vi "Calculation.vi"(0 "Current(i)":dbl, 5 "Voltage(v)":dbl, 7 "Thickness Of Specimen(l)":dbl, 9 "Area of specimen(m2)":dbl, 11 "UPPER(Th-Tc)":dbl, 12 "error constant":errorcluster, 13 "LOWER(Th-Tc)":dbl) -> (4 "Themal Conductivity UPPER":dbl, 6 "Themal Conductivity LOWER":dbl, 10 "Themal Conductivity avg":dbl, 14 "error constant 2":errorcluster)   [LabVIEW 2026]
panel:
  # "Thermal Conductivity= ivl/2A(Th-Tc)"
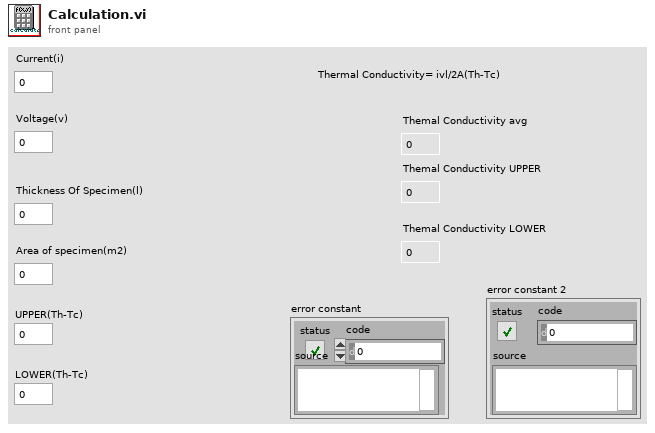
[diagram p1: front panel]
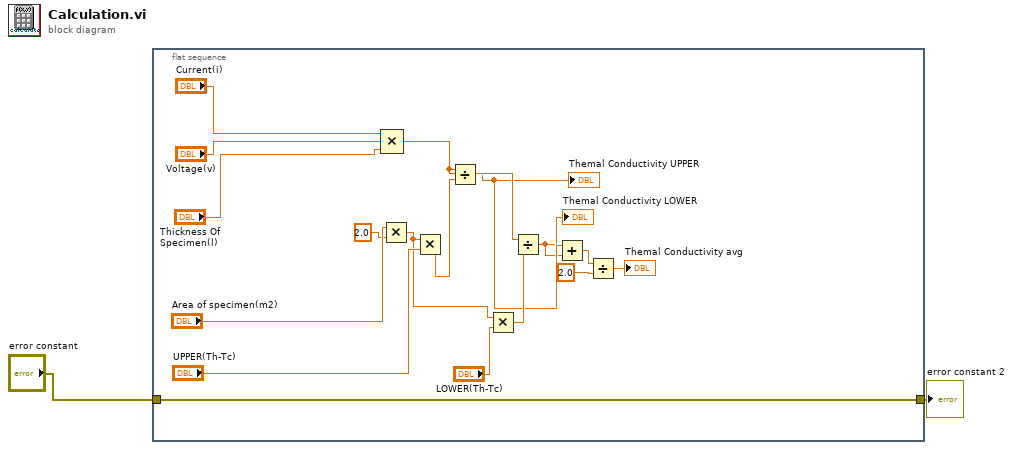
[diagram p0: block diagram]
diagram:
  n1 = flat-sequence {
    tunnel: [w12] -> w1
    tunnel: "error constant" -> [w12]
    frame #0 {
      n2 = Compound Arithmetic op=MULTIPLY("Current(i)", "Voltage(v)", "Thickness Of Specimen(l)") -> (w8:dbl)
      n3 = Multiply(x="Area of specimen(m2)", y=2.0) -> (x*y=w9:dbl)
      n4 = Multiply(x=w9, y="UPPER(Th-Tc)") -> (x*y=w13:dbl)
      n5 = Divide(x=w8, y=w13) -> (x/y=w7:dbl)
      "Themal Conductivity UPPER" <- w7
      n6 = Multiply(x=w9, y="LOWER(Th-Tc)") -> (x*y=w11:dbl)
      n7 = Divide(x=w8, y=w11) -> (x/y=w6:dbl)
      "Themal Conductivity LOWER" <- w6
      n8 = Add(x=w7, y=w6) -> (x+y=w5:dbl)
      n9 = Divide(x=w5, y=2.0) -> (x/y=→"Themal Conductivity avg":dbl)
    }
  }
  "error constant 2" <- w1
